vi "ZM-TST-hardware.vi"() -> (0 "error out":errorcluster, 3 "Pass":bool)   [LabVIEW 2020, in "ZM-TST-tests.lvlib"]
doc: "T3, test of the hardware classes: the simulated hardware's do makes test packages to Communication with data in range that vary between calls; a bare ZM-HW-hardware's do returns 5000. Pass = AND of sim_ok, sim_destination_ok, ranges_ok, varies_ok and placeholder_ok."
uses:
  ZM-TST-tests.lvlib
  hardware/ZM-HW-SIM-simulated_hardware/ZM-HW-SIM-simulated_hardware/ZM-HW-SIM-simulated_hardware.lvclass
  hardware/ZM-HW-hardware/ZM-HW-hardware/ZM-HW-hardware.lvclass
  common/ZM-PC-packages/ZM-PC-package/ZM-PC-package.lvclass
panel:
  out "placeholder_ok":bool
  out "varies_ok":bool
  out "ranges_ok":bool
  out "sim_destination_ok":bool
  out "sim_ok":bool
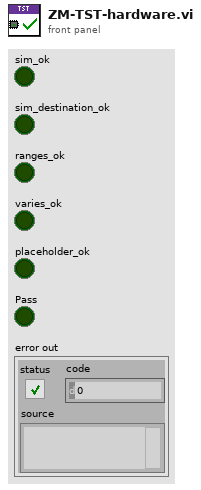
[diagram p1: front panel]
types:
  T1 = cluster{"timestamp":string, "type":string, "destination":string, "data":cluster{"temperature_c":dbl, "sample_index":i32, "duty_percent":u8, "sensor_ok":bool, "status":string}}
  T2 = cluster{"temperature_c":dbl, "sample_index":i32, "duty_percent":u8, "sensor_ok":bool, "status":string}
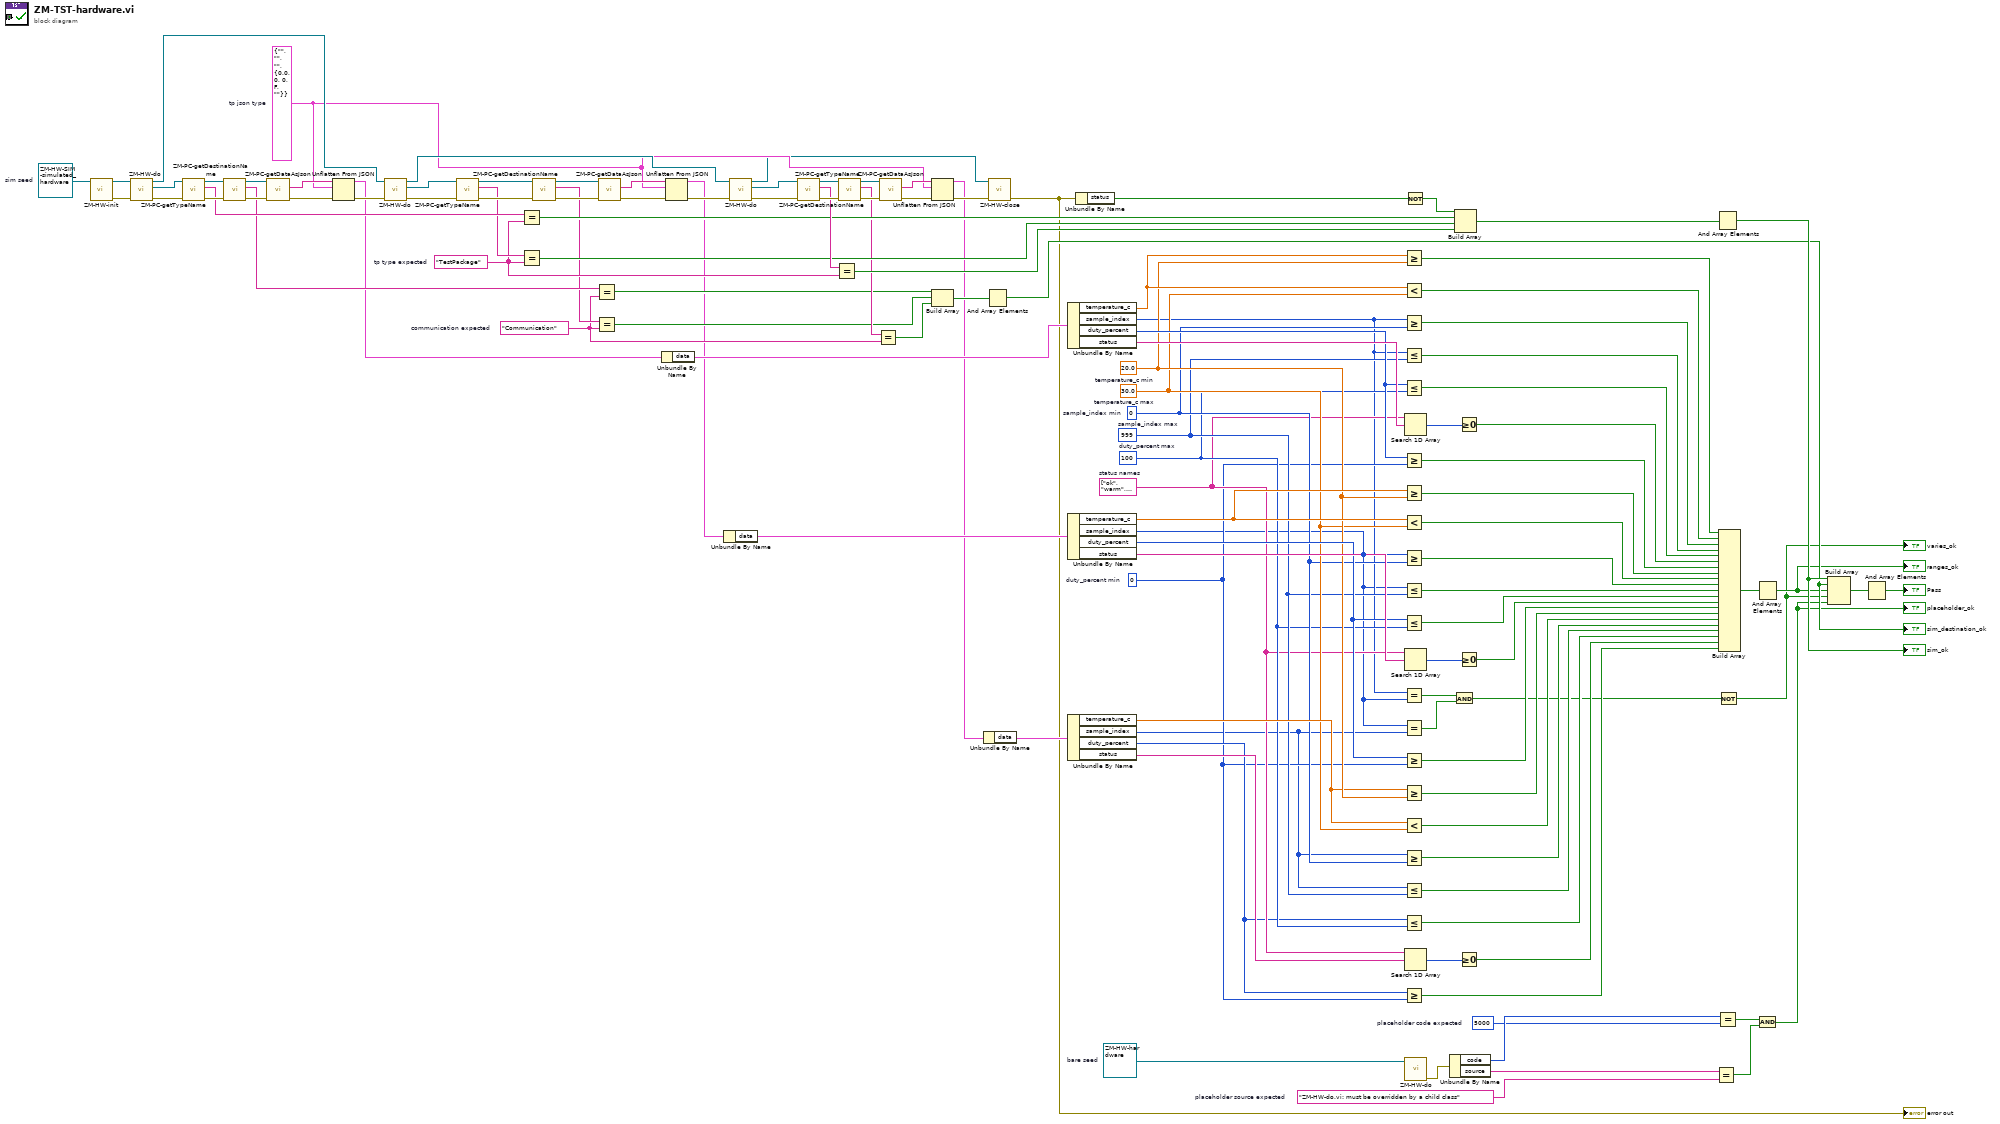
[diagram p0: block diagram]
diagram:
  w45 = u8 0  # duty_percent min
  w11 = "ZM-HW-do.vi: must be overridden by a child class"  # placeholder source expected
  w13 = 5000  # placeholder code expected
  w49 = string[] ["ok", "warm", "cold"]  # status names
  w50 = u8 100  # duty_percent max
  w51 = 999  # sample_index max
  w52 = 0  # sample_index min
  w53 = 30.0  # temperature_c max
  w55 = 20.0  # temperature_c min
  w91 = T1 {"timestamp"="", "type"="", "destination"="", "data"={"temperature_c"=0.0, "sample_index"=0, "duty_percent"=0, "sensor_ok"=FALSE, "status"=""}}  # tp json type
  w74 = "Communication"  # communication expected
  w83 = "TestPackage"  # tp type expected
  w16 = refnum<class "ZM-HW-hardware.lvclass"> refnum  # bare seed
  w121 = refnum<class "ZM-HW-SIM-simulated_hardware.lvclass"> refnum  # sim seed
  n1 = call-dynamic "ZM-HW-init.vi"("ZM-HW-hardware in"=w121) -> ("error out"=w119:errorcluster, "ZM-HW-hardware out"=w120:refnum<class "ZM-HW-SIM-simulated_hardware.lvclass">)  [unwired: 9 in]
  n2 = call-dynamic "ZM-HW-do.vi"("error in (no error)"=w119, "ZM-HW-hardware in"=w120) -> ("error out"=w117:errorcluster, "package"=w118:refnum<class "ZM-PC-package.lvclass">, "ZM-HW-hardware out"=w110:refnum<class "ZM-HW-SIM-simulated_hardware.lvclass">)  [unwired: 7 in]
  n3 = call "ZM-PC-getTypeName.vi"("error in (no error)"=w117, "ZM-PC-package in"=w118) -> ("error out"=w115:errorcluster, "type_name"=w86:string, "ZM-PC-package out"=w116:refnum<class "ZM-PC-package.lvclass">)  [unwired: 7 in]
  n4 = call "ZM-PC-getDestinationName.vi"("error in (no error)"=w115, "ZM-PC-package in"=w116) -> ("error out"=w113:errorcluster, "destination_name"=w77:string, "ZM-PC-package out"=w114:refnum<class "ZM-PC-package.lvclass">)  [unwired: 7 in]
  n5 = call-dynamic "ZM-PC-getDataAsJson.vi"("error in (no error)"=w113, "ZM-PC-package in"=w114) -> ("error out"=w111:errorcluster, "json"=w112:string)  [unwired: 7 in, 1 out]
  n6 = Unflatten From JSON(JSON string=w112, type and defaults=w91, error in (no error)=w111) -> (value=w69:T1, error out=w109:errorcluster)  [unwired: 4 in]
  n7 = call-dynamic "ZM-HW-do.vi"("error in (no error)"=w109, "ZM-HW-hardware in"=w110) -> ("error out"=w107:errorcluster, "package"=w108:refnum<class "ZM-PC-package.lvclass">, "ZM-HW-hardware out"=w100:refnum<class "ZM-HW-SIM-simulated_hardware.lvclass">)  [unwired: 7 in]
  n8 = call "ZM-PC-getTypeName.vi"("error in (no error)"=w107, "ZM-PC-package in"=w108) -> ("error out"=w105:errorcluster, "type_name"=w85:string, "ZM-PC-package out"=w106:refnum<class "ZM-PC-package.lvclass">)  [unwired: 7 in]
  n9 = Equal?(x=w86, y=w83) -> (x = y?=w81:bool)
  n10 = Equal?(x=w85, y=w83) -> (x = y?=w80:bool)
  n11 = call "ZM-PC-getDestinationName.vi"("error in (no error)"=w105, "ZM-PC-package in"=w106) -> ("error out"=w103:errorcluster, "destination_name"=w76:string, "ZM-PC-package out"=w104:refnum<class "ZM-PC-package.lvclass">)  [unwired: 7 in]
  n12 = Equal?(x=w77, y=w74) -> (x = y?=w73:bool)
  n13 = Equal?(x=w76, y=w74) -> (x = y?=w72:bool)
  n14 = call-dynamic "ZM-PC-getDataAsJson.vi"("error in (no error)"=w103, "ZM-PC-package in"=w104) -> ("error out"=w101:errorcluster, "json"=w102:string)  [unwired: 7 in, 1 out]
  n15 = Unbundle By Name(w69) -> ("data"=w68:T2)
  n16 = Unflatten From JSON(JSON string=w102, type and defaults=w91, error in (no error)=w101) -> (value=w63:T1, error out=w99:errorcluster)  [unwired: 4 in]
  n17 = Unbundle By Name(w63) -> ("data"=w62:T2)
  n18 = call-dynamic "ZM-HW-do.vi"("error in (no error)"=w99, "ZM-HW-hardware in"=w100) -> ("error out"=w97:errorcluster, "package"=w98:refnum<class "ZM-PC-package.lvclass">, "ZM-HW-hardware out"=w89:refnum<class "ZM-HW-SIM-simulated_hardware.lvclass">)  [unwired: 7 in]
  n19 = call "ZM-PC-getTypeName.vi"("error in (no error)"=w97, "ZM-PC-package in"=w98) -> ("error out"=w95:errorcluster, "type_name"=w84:string, "ZM-PC-package out"=w96:refnum<class "ZM-PC-package.lvclass">)  [unwired: 7 in]
  n20 = Equal?(x=w84, y=w83) -> (x = y?=w79:bool)
  n21 = call "ZM-PC-getDestinationName.vi"("error in (no error)"=w95, "ZM-PC-package in"=w96) -> ("error out"=w93:errorcluster, "destination_name"=w75:string, "ZM-PC-package out"=w94:refnum<class "ZM-PC-package.lvclass">)  [unwired: 7 in]
  n22 = Equal?(x=w75, y=w74) -> (x = y?=w71:bool)
  n23 = call-dynamic "ZM-PC-getDataAsJson.vi"("error in (no error)"=w93, "ZM-PC-package in"=w94) -> ("error out"=w90:errorcluster, "json"=w92:string)  [unwired: 7 in, 1 out]
  n24 = Unflatten From JSON(JSON string=w92, type and defaults=w91, error in (no error)=w90) -> (value=w57:T1, error out=w88:errorcluster)  [unwired: 4 in]
  n25 = Build Array(w73, w72, w71) -> (w70:bool[])
  n26 = Unbundle By Name(w57) -> ("data"=w56:T2)
  n27 = And Array Elements(Boolean array=w70) -> (logical AND=w6:bool)
  "sim_destination_ok" <- w6
  n28 = call-dynamic "ZM-HW-close.vi"("error in (no error)"=w88, "ZM-HW-hardware in"=w89) -> ("error out"=w1:errorcluster)  [unwired: 8 in, 1 out]
  "error out" <- w1
  n29 = Unbundle By Name(w68) -> ("temperature_c"=w67:dbl, "sample_index"=w22:i32, "duty_percent"=w64:u8, "status"=w66:string)
  n30 = Unbundle By Name(w62) -> ("temperature_c"=w61:dbl, "sample_index"=w21:i32, "duty_percent"=w58:u8, "status"=w60:string)
  n31 = Unbundle By Name(w56) -> ("temperature_c"=w54:dbl, "sample_index"=w20:i32, "duty_percent"=w46:u8, "status"=w48:string)
  n32 = Unbundle By Name(w1) -> ("status"=w87:bool)
  n33 = Greater Or Equal?(x=w67, y=w55) -> (x >= y?=w44:bool)
  n34 = Less?(x=w67, y=w53) -> (x < y?=w43:bool)
  n35 = Greater Or Equal?(x=w22, y=w52) -> (x >= y?=w42:bool)
  n36 = Less Or Equal?(x=w22, y=w51) -> (x <= y?=w41:bool)
  n37 = Less Or Equal?(x=w64, y=w50) -> (x <= y?=w40:bool)
  n38 = Greater Or Equal?(x=w64, y=w45) -> (x >= y?=w38:bool)
  n39 = Greater Or Equal?(x=w61, y=w55) -> (x >= y?=w37:bool)
  n40 = Less?(x=w61, y=w53) -> (x < y?=w36:bool)
  n41 = Greater Or Equal?(x=w21, y=w52) -> (x >= y?=w35:bool)
  n42 = Less Or Equal?(x=w21, y=w51) -> (x <= y?=w34:bool)
  n43 = Less Or Equal?(x=w58, y=w50) -> (x <= y?=w33:bool)
  n44 = Equal?(x=w22, y=w21) -> (x = y?=w19:bool)
  n45 = Equal?(x=w21, y=w20) -> (x = y?=w18:bool)
  n46 = Greater Or Equal?(x=w58, y=w45) -> (x >= y?=w31:bool)
  n47 = Greater Or Equal?(x=w54, y=w55) -> (x >= y?=w30:bool)
  n48 = Less?(x=w54, y=w53) -> (x < y?=w29:bool)
  n49 = Greater Or Equal?(x=w20, y=w52) -> (x >= y?=w28:bool)
  n50 = Less Or Equal?(x=w20, y=w51) -> (x <= y?=w27:bool)
  n51 = Less Or Equal?(x=w46, y=w50) -> (x <= y?=w26:bool)
  n52 = Greater Or Equal?(x=w46, y=w45) -> (x >= y?=w24:bool)
  n53 = Not(x=w87) -> (.not. x?=w82:bool)
  n54 = Search 1D Array(1D array=w49, element=w66) -> (index of element=w65:i32)  [unwired: 1 in]
  n55 = Search 1D Array(1D array=w49, element=w60) -> (index of element=w59:i32)  [unwired: 1 in]
  n56 = Search 1D Array(1D array=w49, element=w48) -> (index of element=w47:i32)  [unwired: 1 in]
  n57 = call-dynamic "ZM-HW-do.vi"("ZM-HW-hardware in"=w16) -> ("error out"=w15:errorcluster)  [unwired: 8 in, 2 out]
  n58 = Unbundle By Name(w15) -> ("code"=w14:i32, "source"=w12:string)
  n59 = And(x=w19, y=w18) -> (x .and. y?=w17:bool)
  n60 = Build Array(w82, w81, w80, w79) -> (w78:bool[])
  n61 = Greater Or Equal To 0?(x=w65) -> (x >= 0?=w39:bool)
  n62 = Greater Or Equal To 0?(x=w59) -> (x >= 0?=w32:bool)
  n63 = Greater Or Equal To 0?(x=w47) -> (x >= 0?=w25:bool)
  n64 = Equal?(x=w12, y=w11) -> (x = y?=w9:bool)
  n65 = And Array Elements(Boolean array=w78) -> (logical AND=w7:bool)
  "sim_ok" <- w7
  n66 = Equal?(x=w14, y=w13) -> (x = y?=w10:bool)
  n67 = Not(x=w17) -> (.not. x?=w4:bool)
  "varies_ok" <- w4
  n68 = Build Array(w44, w43, w42, w41, w40, w39, w38, w37, w36, w35, w34, w33, w32, w31, w30, w29, w28, w27, w26, w25, w24) -> (w23:bool[])
  n69 = And Array Elements(Boolean array=w23) -> (logical AND=w5:bool)
  "ranges_ok" <- w5
  n70 = And(x=w10, y=w9) -> (x .and. y?=w3:bool)
  "placeholder_ok" <- w3
  n71 = Build Array(w7, w6, w5, w4, w3) -> (w8:bool[])
  n72 = And Array Elements(Boolean array=w8) -> (logical AND=→"Pass":bool)
